vi "FuncVI2-CallLevel.vi"(4 "CSE RefNum":T1, 5 "InstanceRef":T3, 9 "arg list":T2[](array[typedef]) {"num" format="%.2f"}) -> (0 "error out":bool, 3 "result":T2 {"num" format="%.2f"})   [LabVIEW 2021]
doc: "::: CalcExpress Toolkit :::\nCopyright (c) 2000-2026 Konstantin Shifershteyn. All rights reserved."
uses:
  cetypes.llb/CalcExpress Function Argument Info.ctl
  cetypes.llb/CalcExpress Instance RefNum.ctl
  cse.llb/CSE Instance RefNum.ctl
panel:
  in  "max arg num":i32
  in  "min arg num":i32
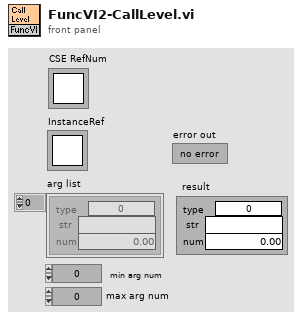
[diagram p1: front panel]
types:
  T1 = typedef "CSE Instance RefNum.ctl" = refnum<k1>
  T2 = typedef "CalcExpress Function Argument Info.ctl" = cluster{"type":u32, "str":string, "num":dbl}
  T3 = typedef "CalcExpress Instance RefNum.ctl" = refnum<k1>
  T4 = enum32{"String", "DBL Number", "identifier", "1D Array of DBL", "2D Array of DBL", "CDB Number", "1D Array of CDB", "2D Array of CDB", "1D Array of String", "2D Array of String", "Unknown data type"}
  T5 = cluster{"level":i32, "Caller CSE RefNum":T1, "Callee CSE RefNum":T1}
  T6 = cluster{"type: use this constant to specify a predefined type code":enum32{"String", "DBL Number", "identifier", "1D Array of DBL", "2D Array of DBL", "CDB Number", "1D Array of CDB", "2D Array of CDB", "1D Array of String", "2D Array of String", "Unknown data type"}, string, dbl}
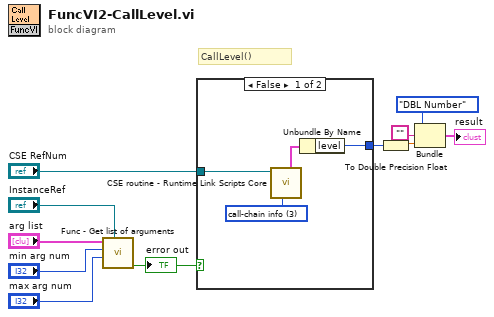
[diagram p0: block diagram]
diagram:
  # "CallLevel()"
  n1 = call "Func - Get list of arguments.vi"("InstanceRef"="InstanceRef", "max arg num"="max arg num", "min arg num"="min arg num", "arg list"="arg list") -> ("error out"=w5:bool)  [unwired: 4 in, 3 out]
  "error out" <- w5
  n2 = case shown="False" w5 {
    tunnel: [w13 _] -> w3
    tunnel: "CSE RefNum" -> [w12 _]
    frame False {
      w15 = 3 items=["save vi path", "link to caller", "delink of caller", "call-chain info"] ("action")
      n3 = call "CSE routine - Runtime Link Scripts Core.vi"("action"=w15, "CSE RefNum"=w12) -> ("call-chain info"=w14:T5)  [unwired: 4 in, 5 out]
      n4 = Unbundle By Name(w14) -> ("level"=w13:i32)
    }
    frame True {
    }
  }
  n5 = To Double Precision Float(number=w3) -> (double precision float=w2:dbl)
  n6 = Bundle("type: use this constant to specify a predefined type code"=T4."DBL Number", "", w2) -> (→"result":T6)  [unwired: 1 in]
